vi "Set Description.vi"(8 "error in":errorcluster, 11 "ILabVIEWFile in":refnum<class "Virtual Instrument.lvclass">) -> (0 "error out":errorcluster, 3 "ILabVIEWFile out":refnum<class "Virtual Instrument.lvclass">)   [LabVIEW 2026, in "Virtual Instrument.lvclass"]
doc: "Set description of labview file (vi or type definition)."
uses:
  Virtual Instrument.lvclass
  LabVIEW File/LabVIEW File.lvclass/LabVIEW File.ctl
  Virtual Instrument.lvclass/Virtual Instrument.ctl
  LabVIEW File/Read VI Reference.vi
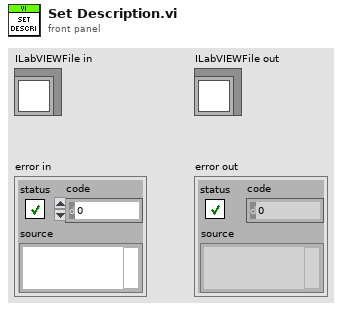
[diagram p1: front panel]
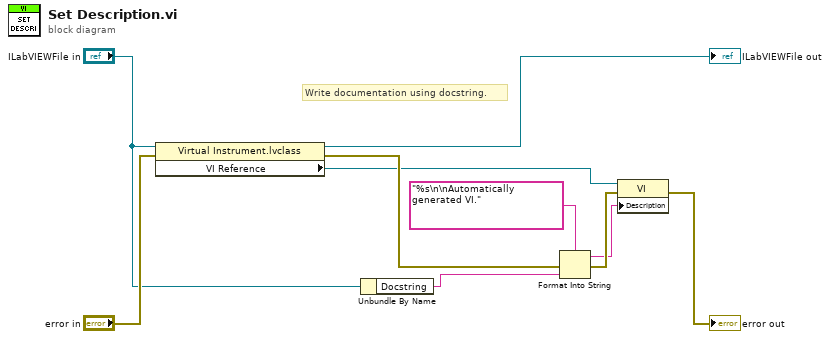
[diagram p0: block diagram]
diagram:
  # "Write documentation using docstring."
  n1 = property class="Virtual Instrument.lvclass"(reference="ILabVIEWFile in", error in="error in") -> (reference out=→"ILabVIEWFile out":refnum<class "Virtual Instrument.lvclass">, error out=w7:errorcluster, "VI Reference"=w1:refnum<vi>)
  n2 = Unbundle By Name("ILabVIEWFile in") -> ("Docstring"=w5:string)
  n3 = Format Into String(format string="%s\n\nAutomatically generated VI.", error in=w7, w5) -> (resulting string=w4:string, error out=w10:errorcluster)  [unwired: 1 in]
  n4 = property class="VI"(reference=w1, error in=w10, "Description"=w4) -> (error out=→"error out":errorcluster)  [unwired: 1 out]
